vi "populate_map.vi"(8 "error in (no error)":errorcluster, 10 "variable_info_in":T3, 11 "IO_variable_map_in":T1[](array[typedef])) -> (0 "error out":errorcluster, 3 "IO_variable_map_out":T1[](array[typedef]))   [LabVIEW 2015, in "Scan Engine runtime.lvclass"]
uses:
  Scan Engine runtime.lvclass
  Custom Ctrls/Index Map.ctl
  <vilib>/NI/Tag Bus/tag/Data Type.ctl
  Custom Ctrls/IO_index_map.ctl
  <vilib>/NI/Tag Bus/tag/tag descriptor.lvclass
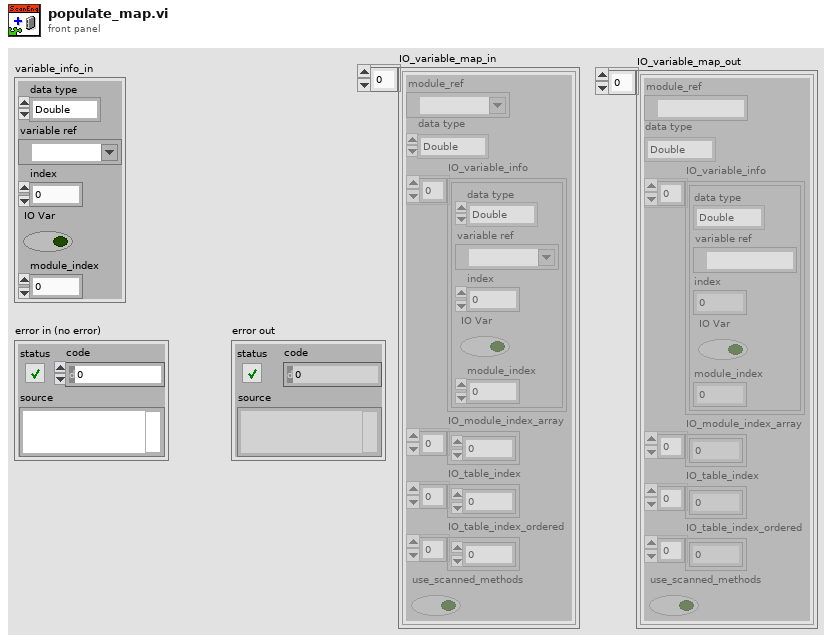
[diagram p1: front panel]
types:
  T1 = typedef "Scan Engine runtime.lvclass/IO_index_map.ctl" = cluster{"module_ref":refnum<k21>, "data type":T2, "IO_variable_info":T3[], "IO_module_index_array":i32[], "IO_table_index":i32[], "IO_table_index_ordered":i32[], "use_scanned_methods":bool}
  T2 = typedef "tag bus.lvlib/tag descriptor.lvclass/Data Type.ctl" = enum16{"Double", "Single", "I64", "I32", "I16", "I8", "U64", "U32", "U16", "U8", "Boolean", "String", "Array of Double", "Array of Single", "Array of I64", "Array of I32", "Array of I16", "Array of I8", "Array of U64", "Array of U32", "Array of U16", "Array of U8", "Array of Boolean", "Array of String"}
  T3 = typedef "Scan Engine runtime.lvclass/Index Map.ctl" = cluster{"data type":T2, "variable ref":refnum<k21>, "index":i32, "IO Var":bool, "module_index":i32}
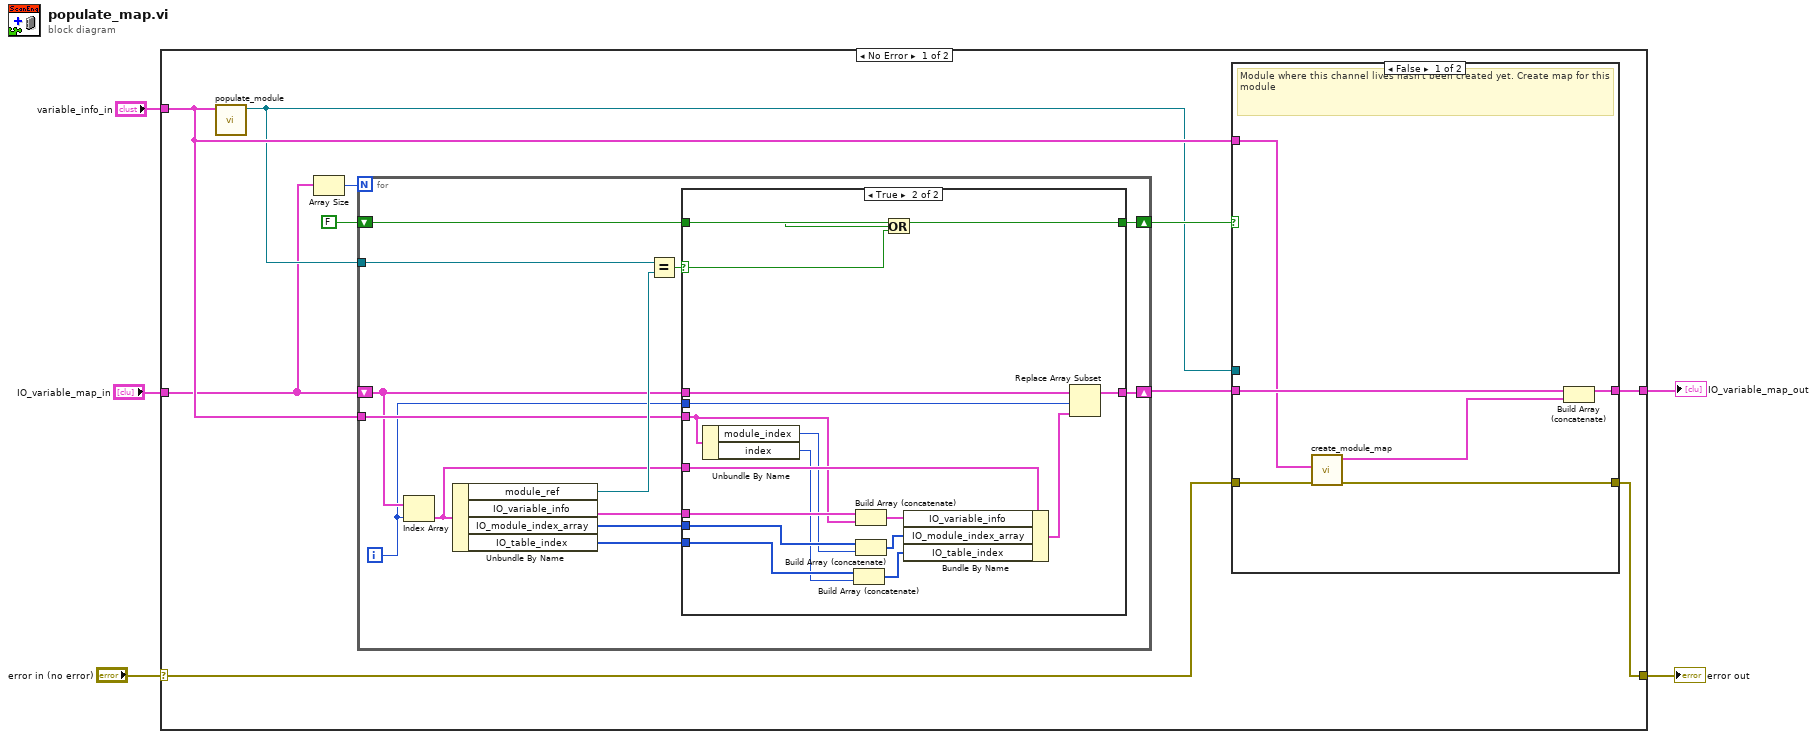
[diagram p0: block diagram]
diagram:
  n1 = case shown="No Error" "error in (no error)" {
    selector: "error in (no error)" -> [w7 w57]
    tunnel: "variable_info_in" -> [w11 _]
    tunnel: "IO_variable_map_in" -> [w9 w56]
    tunnel: [w8 w56] -> w1
    tunnel: [w6 w57] -> w2
    frame No Error {
      n2 = call "populate_module.vi"("variable_info_in"=w11) -> ("Module"=w10:refnum<k21>)  [unwired: 10 in]
      n3 = Array Size(array=w9) -> (size(s)=w15:i32)
      n4 = for {
        N: w15 -> [_]
        tunnel: w10 -> [w36]
        tunnel: w11 -> [w33]
        shift-right: [w29] -> w12
        shift-left: w9 -> [w32]
        shift-right: [w26] -> w13
        shift-left: FALSE -> [w27]
        i -> [w30]
        n5 = Index Array(array=w32, index=w30) -> (element=w31:T1)
        n6 = Unbundle By Name(w31) -> ("module_ref"=w35:refnum<k21>, "IO_variable_info"=w34:T3[], "IO_module_index_array"=w25:i32[], "IO_table_index"=w24:i32[])
        n7 = Equal?(x=w36, y=w35) -> (x = y?=w28:bool)
        n8 = case shown="True" w28 {
          selector: w28 -> [_ w48]
          tunnel: w34 -> [_ w55]
          tunnel: w33 -> [_ w44]
          tunnel: w32 -> [w38 w54]
          tunnel: w31 -> [_ w53]
          tunnel: w30 -> [_ w52]
          tunnel: [w38 w51] -> w29
          tunnel: w27 -> [w37 w49]
          tunnel: [w37 w47] -> w26
          tunnel: w25 -> [_ w45]
          tunnel: w24 -> [_ w40]
          frame False {
          }
          frame True {
            n9 = Unbundle By Name(w44) -> ("module_index"=w43:i32, "index"=w39:i32)
            n10 = Build Array (concatenate)(w40, w39) -> (w41:i32[])
            n11 = Build Array (concatenate)(w55, w44) -> (w46:T3[])
            n12 = Build Array (concatenate)(w45, w43) -> (w42:i32[])
            n13 = Or(x=w49, y=w48) -> (x .or. y?=w47:bool)
            n14 = Bundle By Name(cluster=w53, "IO_variable_info"=w46, "IO_module_index_array"=w42, "IO_table_index"=w41) -> (w50:T1)
            n15 = Replace Array Subset(array=w54, new element=w50, index=w52) -> (w51:T1[])
          }
        }
      }
      n16 = case shown="False" w13 {
        tunnel: w12 -> [w21 w23]
        tunnel: [w20 w23] -> w8
        tunnel: w10 -> [_ _]
        tunnel: w11 -> [w18 _]
        tunnel: w7 -> [w19 w22]
        tunnel: [w16 w22] -> w6
        frame False {
          # "Module where this channel lives hasn't been created yet. Create map for this module"
          n17 = call "create_module_map.vi"("error in (no error)"=w19, "variable_info_in"=w18) -> ("error out"=w16:errorcluster, "IO_variable_map"=w17:T1[])  [unwired: 8 in]
          n18 = Build Array (concatenate)(w21, w17) -> (w20:T1[])
        }
        frame True {
          # "Channel was added in previously created module"
        }
      }
    }
    frame Error {
    }
  }
  "IO_variable_map_out" <- w1
  "error out" <- w2
